vi "configuration UI.vi"() -> ()   [LabVIEW 2013, in "TEC editor node.lvclass"]
uses:
  TEC editor node.lvclass
  <vilib>/NI/Configuration Framework/Node/NodeRef.ctl
  <vilib>/NI/Configuration Framework/Node/NISE_CEF_Node.lvclass
  <vilib>/NI/AMC/Message Queue.ctl
  <vilib>/NI/AMC/Message.ctl
  <vilib>/NI/Tools/Keyed Array/KeyedArray.ctl
  <vilib>/NI/Configuration Framework/Node/UserEventRef.ctl
  <vilib>/NI/Configuration Framework/Controls/EventCluster.ctl
  <vilib>/NI/DCAF UI Toolkit/Controls/Move One Right.ctl
  <vilib>/NI/DCAF UI Toolkit/Controls/Move One Left.ctl
  configuration/TEC configuration.lvclass
  <vilib>/Utility/miscctls.llb/LVRowAndColumnTypeDef.ctl
  <vilib>/Utility/miscctls.llb/LVPositionTypeDef.ctl
  configuration/TEC configuration.lvclass/TEC configuration.ctl
  TEC editor node.lvclass/TEC editor node.ctl
  <vilib>/NI/Tag Bus/tag/Data Type.ctl
  <vilib>/NI/Tag Bus Module Framework/channel/channel classification.ctl
  <vilib>/NI/Tag Bus Module Framework/channel/TBM channel.lvclass/TBM channel.ctl
  <vilib>/NI/Configuration Framework/serializable configuration/NISE_CEF_serializable configuration.lvclass/NISE_CEF_serializable configuration.ctl
  <vilib>/NI/Tag Bus/tag/tag descriptor.lvclass/tag descriptor.ctl
  configuration/Write receive on port.vi
  configuration/Write send to port.vi
  configuration/Write send from port.vi
  configuration/Write send to address.vi
  configuration/Write estimated array size.vi
  configuration/Read receive on port.vi
  configuration/Read send from port.vi
  configuration/Read send to address.vi
  configuration/Read send to port.vi
  configuration/Read estimated array size.vi
  <vilib>/NI/DCAF/Tag Editor Core/Configuration Editor/Classes/Module editor node/Read display name.vi
  <vilib>/Utility/LVClass/Get LV Class Name.vi
  <vilib>/NI/Configuration Framework/error generator/NISE_error generator.vi
  <vilib>/NI/Configuration Framework/serializable configuration/NISE_CEF_serializable configuration.lvclass
  <vilib>/NI/DCAF/Tag Editor Core/Configuration Editor/Classes/Module editor node/module editor node.lvclass
  <vilib>/NI/Configuration Framework/NISE_CEF_TreeControl.lvlib
  <vilib>/NI/Tag Bus/tag/tag descriptor.lvclass
  <vilib>/NI/Module Execution Interface/Engine Configuration/engine configuration.lvclass
  <vilib>/NI/Tag Bus Module Framework/channel/TBM channel.lvclass
  <vilib>/NI/DCAF/Tag Editor Core/Configuration Editor/Classes/Engine Parent/Engine Parent Editor Node.lvclass
  <vilib>/NI/DCAF UI Toolkit/Controls/DCAF UI Elements.lvlib
  <vilib>/NI/Tools/Keyed Array/Tools_KeyedArray.lvlib
  <vilib>/NI/AMC/AMC.lvlib
panel:
  in  "Tab Control":T1(tab)
  out "Guid":string
  in  "unpair":bool
  out "Paired with":string
  in  "pair":bool
  in  "Pairing Options":i32(listbox)
  in  "Filtering":string
  in  "remove to":T2
  in  "add to":T3
  in  "toExtList":i32(listbox)
  in  "fromExternallist":i32(listbox)
  in  "avail tags":i32(listbox)=-1
  in  "Estimated Received Array Size (bytes)":u16
  in  "receive on port":u16
  in  "send from port":u16
  in  "send to address":string
  in  "send to port":u16
  in  "user event":T4
  in  "main queue":T5
  in  "node ref":T6
  # "UDP Port Settings"
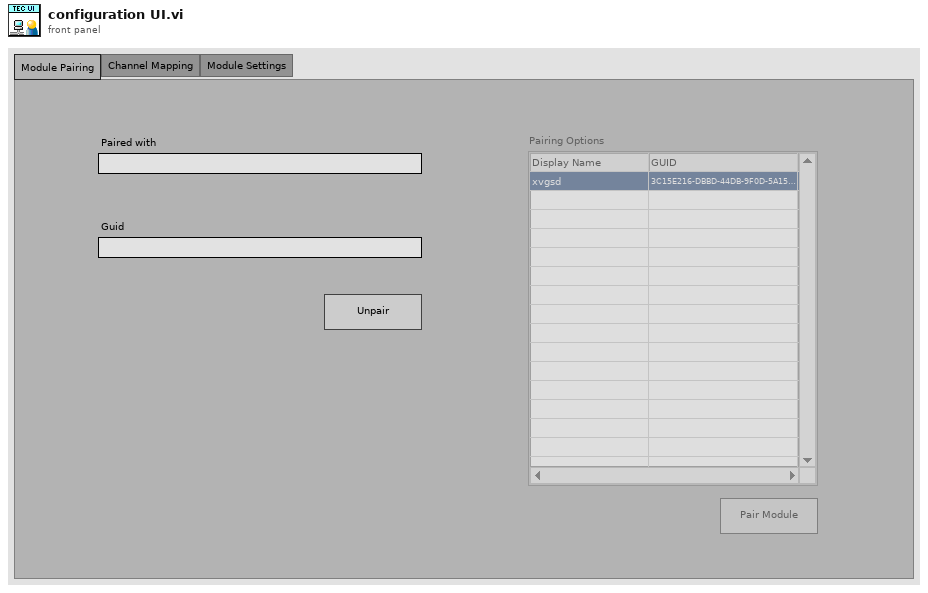
[diagram p1: front panel]
types:
  T1 = enum32{"Module Pairing", "Channel Mapping", "Module Settings"}
  T2 = typedef "DCAF UI Elements.lvlib/Move One Left.ctl" = bool
  T3 = typedef "DCAF UI Elements.lvlib/Move One Right.ctl" = bool
  T4 = typedef "NISE_CEF_Node.lvclass/UserEventRef.ctl" = refnum<user-event>
  T5 = typedef "AMC.lvlib/Message Queue.ctl" = refnum<queue>
  T6 = typedef "NISE_CEF_Node.lvclass/NodeRef.ctl" = refnum<data-value>
  T7 = typedef "LVPositionTypeDef.ctl" = cluster{"Left":i32, "Top":i32}
  T8 = typedef "LVRowAndColumnTypeDef.ctl" = cluster{"Row":i32, "Column":i32}
  T9 = typedef "NISE_CEF_TreeControl.lvlib/EventCluster.ctl" = cluster{"command":string, "data":string}
  T10 = typedef "TBM channel.lvclass/channel classification.ctl" = enum16{"input data", "output data", "processing parameter", "processing result"}
  T11 = typedef "tag bus.lvlib/tag descriptor.lvclass/Data Type.ctl" = enum16{"Double", "Single", "I64", "I32", "I16", "I8", "U64", "U32", "U16", "U8", "Boolean", "String", "Array of Double", "Array of Single", "Array of I64", "Array of I32", "Array of I16", "Array of I8", "Array of U64", "Array of U32", "Array of U16", "Array of U8", "Array of Boolean", "Array of String"}
  T12 = typedef "TEC editor node.lvclass/pair information.ctl" = cluster{"paired guid":string}
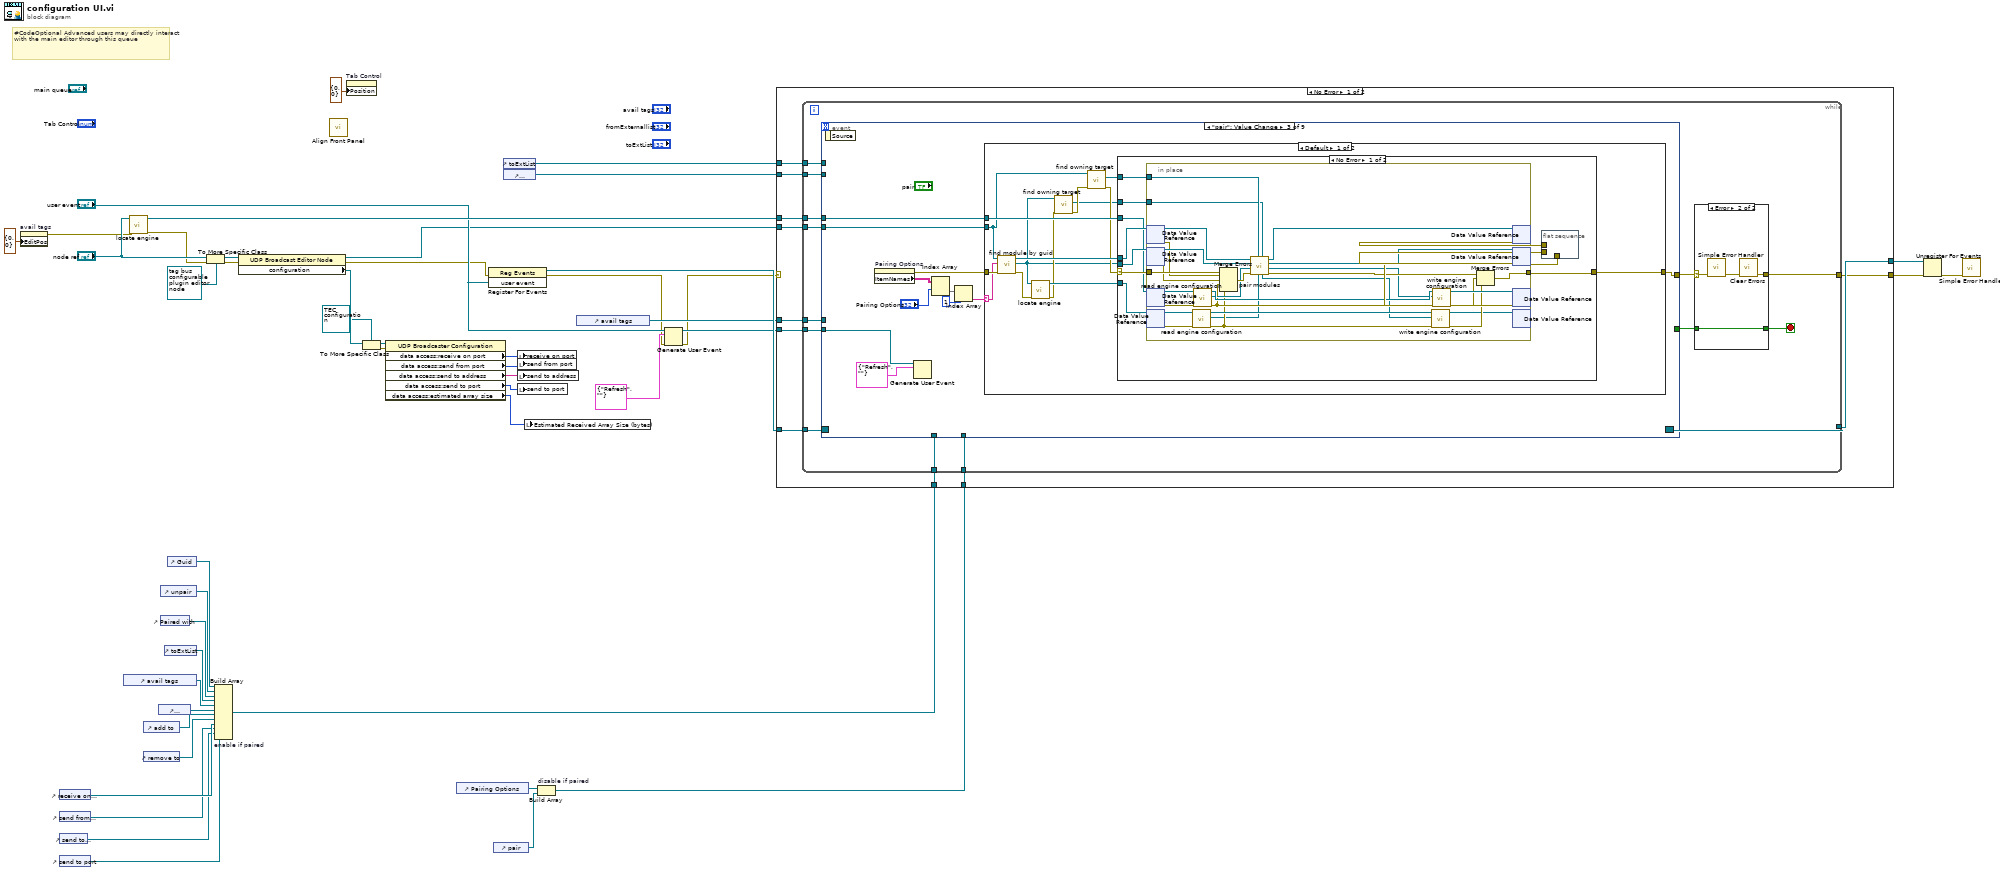
[diagram p0: block diagram]
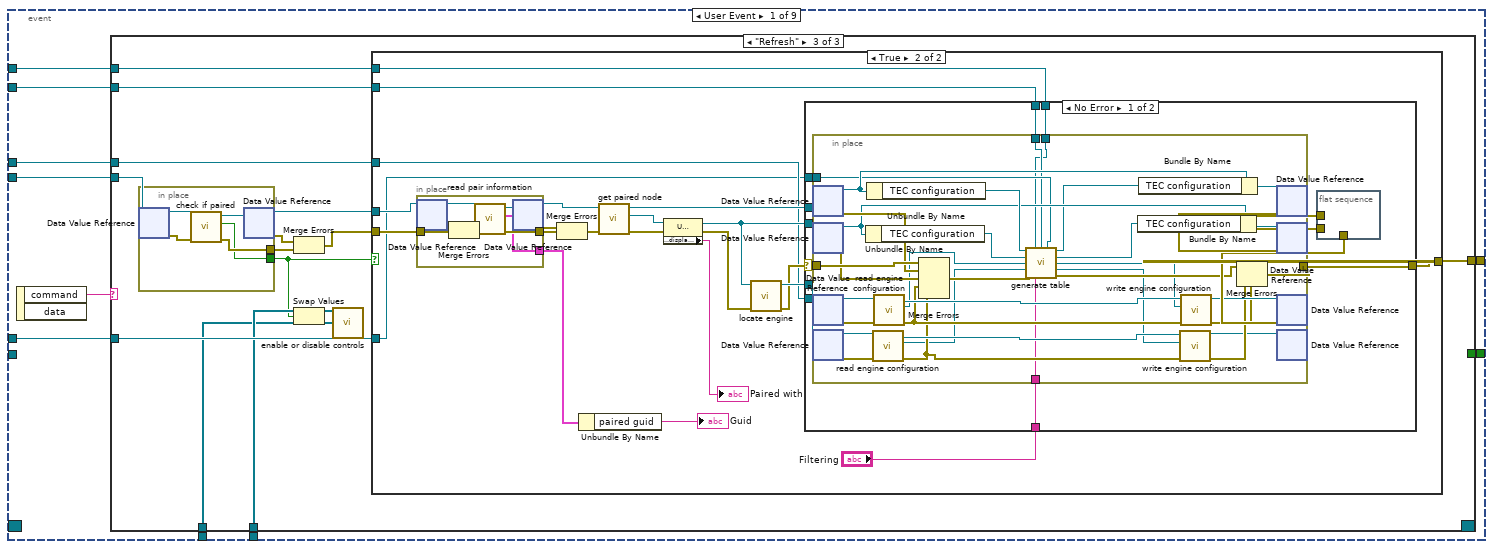
[diagram p3: hidden frame]
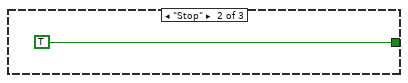
[diagram p5: hidden frame]
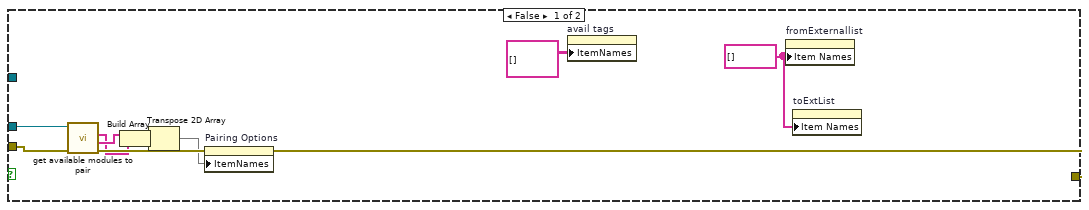
[diagram p6: hidden frame]
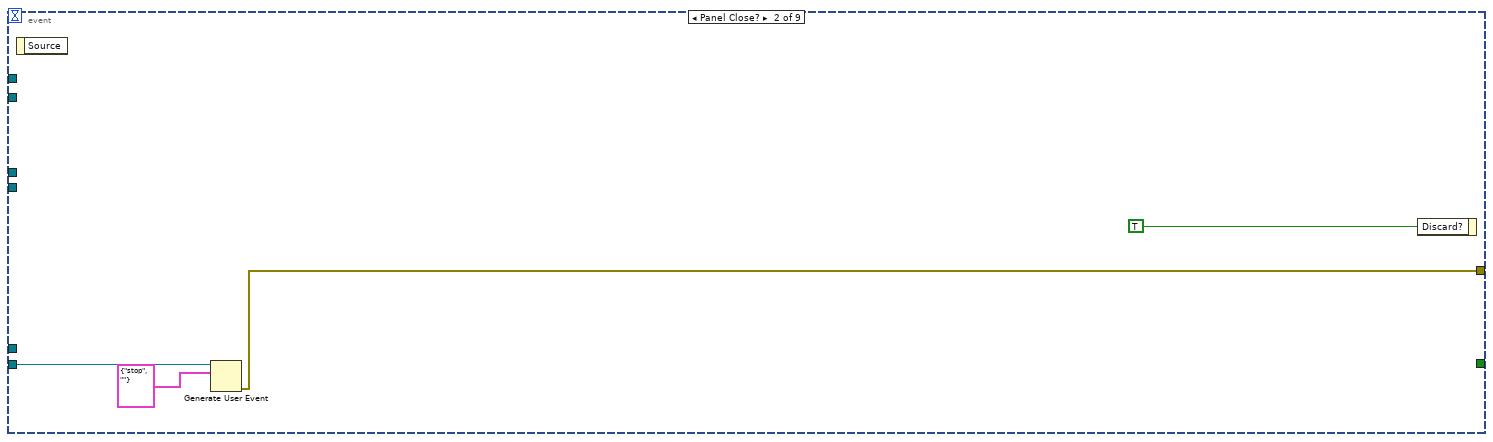
[diagram p8: hidden frame]
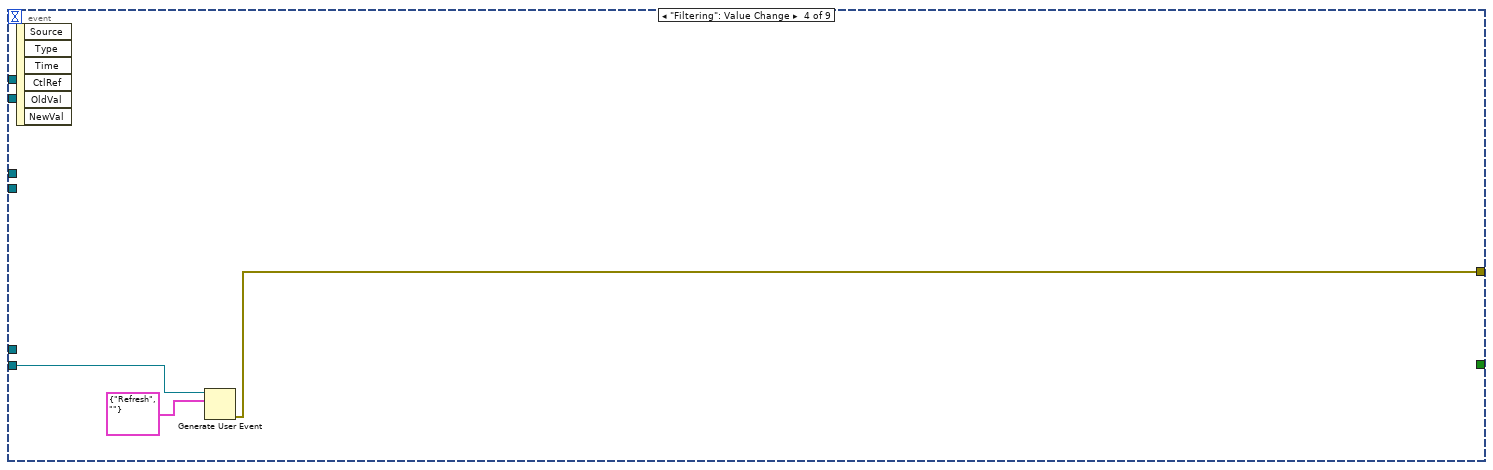
[diagram p11: hidden frame]
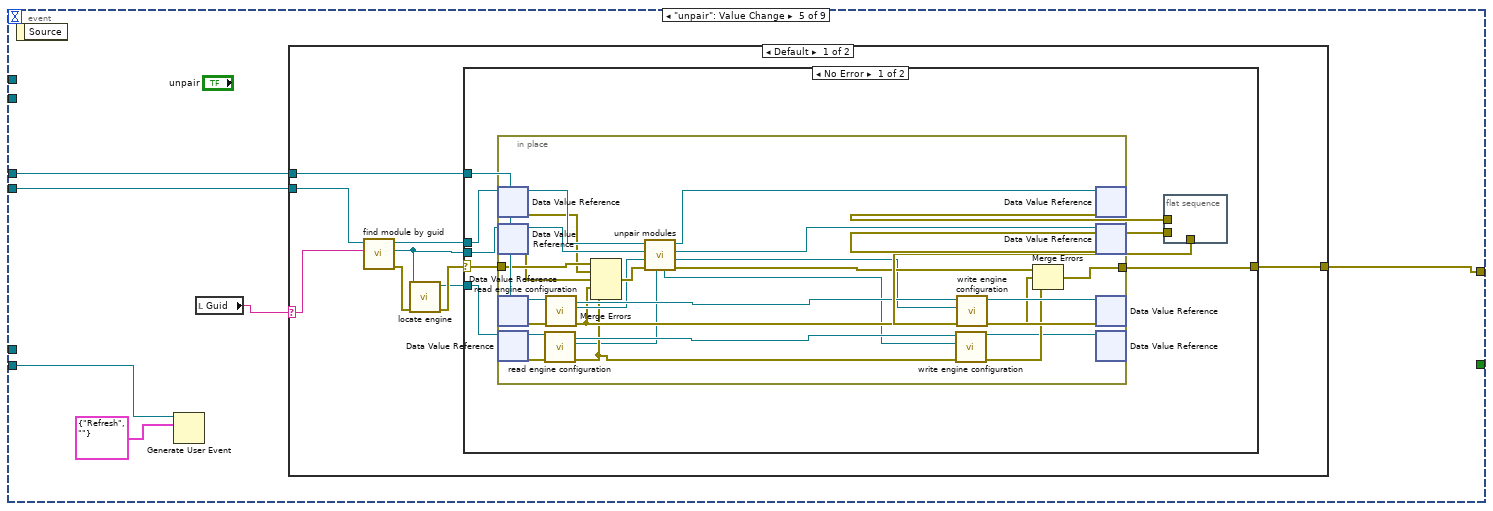
[diagram p12: hidden frame]
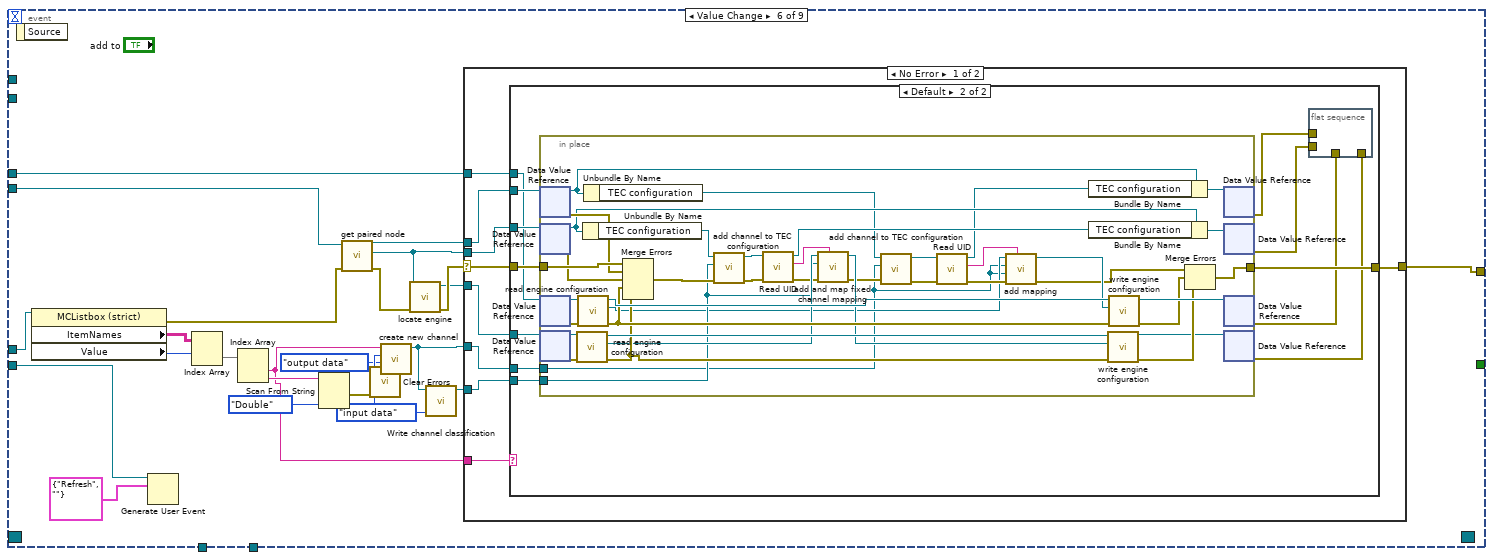
[diagram p15: hidden frame]
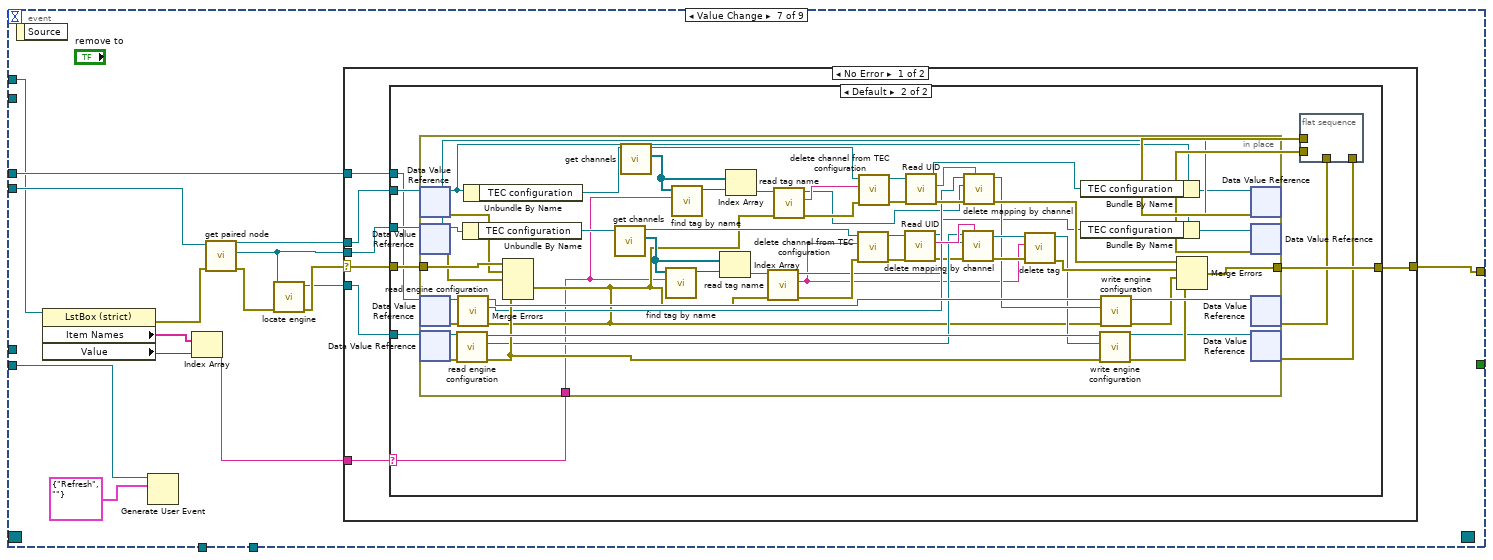
[diagram p18: hidden frame]
diagram:
  # "#CodeOptional Advanced users may directly interact with the main editor through this queue"
  n1 = property on="avail tags" class="MCListbox (strict)"("EditPos"=T8 {"Row"=0, "Column"=0} ("Edit Position")) -> (error out=w4:errorcluster)  [unwired: 2 in, 1 out]
  n2 = control-ref of="receive on port"() -> (w8:refnum<vi>)
  n3 = control-ref of="send from port"() -> (w7:refnum<vi>)
  n4 = control-ref of="send to address"() -> (w6:refnum<vi>)
  n5 = control-ref of="send to port"() -> (w5:refnum<vi>)
  n6 = control-ref of="avail tags"() -> (w29:refnum<vi>)
  n7 = call <vilib>:"locate engine.vi"("error in"=w4, "component"="node ref") -> ("error out"=w34:errorcluster, "engine"=w42:refnum<data-value>)  [unwired: 8 in]
  n8 = control-ref of="add to"() -> (w26:refnum<vi>)
  n9 = control-ref of="remove to"() -> (w27:refnum<vi>)
  n10 = control-ref of="fromExternallist"() -> (w28:refnum<vi>)
  n11 = control-ref of="unpair"() -> (w32:refnum<vi>)
  n12 = control-ref of="Paired with"() -> (w33:refnum<vi>)
  n13 = control-ref of="toExtList"() -> (w30:refnum<vi>)
  n14 = control-ref of="Guid"() -> (w31:refnum<vi>)
  n15 = To More Specific Class(target class=refnum<data-value> refnum ("data value reference"), reference="node ref", error in=w34) -> (specific class reference=w18:refnum<data-value>, error out=w44:errorcluster)
  n16 = Build Array "enable if paired"(w31, w32, w33, w30, w29, w28, w26, w27, w8, w7, w6, w5) -> (w24:refnum<vi>[])
  n17 = property class="UDP Broadcast Editor Node"(reference=w18, error in=w44) -> (reference out=w17:refnum<data-value>, error out=w19:errorcluster, "configuration"=w12:refnum<class "NISE_CEF_serializable configuration.lvclass">)
  n18 = call <vilib>:"Align Front Panel.vi"() -> ()  [unwired: 10 in, 2 out]
  n19 = property on="Tab Control" class="TabCtl (strict)"("Position"=T7 {"Left"=0, "Top"=0}) -> ()  [unwired: 2 in, 2 out]
  n20 = To More Specific Class(target class=refnum<class "TEC configuration.lvclass"> refnum ("UDP Broadcaster Configuration"), reference=w12) -> (specific class reference=w11:refnum<class "TEC configuration.lvclass">, error out=w10:errorcluster)  [unwired: 1 in]
  n21 = property class="UDP Broadcaster Configuration"(reference=w11, error in=w10) -> ("data access:receive on port"=w13:u16, "data access:send from port"=w14:u16, "data access:send to address"=w15:string, "data access:send to port"=w16:u16, "data access:estimated array size"=w2:u16)  [unwired: 2 out]
  n22 = control-ref of="Pairing Options"() -> (w25:refnum<vi>)
  n23 = register-events(error in=w19, "user event") -> (reference out=w48:refnum<event-registration>, error out=w21:errorcluster)  [unwired: 1 in]
  n24 = control-ref of="pair"() -> (w22:refnum<vi>)
  n25 = control-ref of="toExtList"() -> (w40:refnum<vi>)
  n26 = control-ref of="fromExternallist"() -> (w20:refnum<vi>)
  n27 = local write "receive on port"(w13) -> ()
  n28 = local write "send from port"(w14) -> ()
  n29 = local write "send to address"(w15) -> ()
  n30 = local write "send to port"(w16) -> ()
  n31 = local write "Estimated Received Array Size (bytes)"(w2) -> ()
  n32 = Build Array "disable if paired"(w25, w22) -> (w23:refnum<vi>[])
  n33 = control-ref of="avail tags"() -> (w41:refnum<vi>)
  n34 = Generate User Event(user event="user event", event data cluster=T9 {"command"="Refresh", "data"=""} ("event data"), error in=w21) -> (user event out=w38:T4, error out=w36:errorcluster)  [unwired: 1 in]
  n35 = case shown="No Error" w36 {
    selector: w36 -> [_ w540]
    tunnel: w48 -> [w59 w539]
    tunnel: [w58 w539] -> w47
    tunnel: [w57 w540] -> w46
    tunnel: w17 -> [w56 _]
    tunnel: w42 -> [w55 _]
    tunnel: w41 -> [w54 _]
    tunnel: w40 -> [w53 _]
    tunnel: w38 -> [w52 _]
    tunnel: w24 -> [w51 _]
    tunnel: w23 -> [w50 _]
    tunnel: w20 -> [w49 _]
    frame No Error {
      n36 = while {
        tunnel: w59 -> [w73]
        tunnel: [w72] -> w58
        tunnel: w56 -> [w67]
        tunnel: w55 -> [w66]
        tunnel: w52 -> [w65]
        tunnel: w54 -> [w64]
        tunnel: w53 -> [w63]
        tunnel: [w68] -> w57
        tunnel: w51 -> [w62]
        tunnel: w50 -> [w61]
        tunnel: w49 -> [w60]
        stop <- w70 stop-if-true
        n37 = event shown="[2] \"pair\": Value Change" {
          selector: w73 -> [_ _ _ _ _ _ _ _ _]
          dyn-events: [_ _ _ _ _ _ _ _ _] -> w72
          timeout: _ -> [_ _ _ _ _ _ _ _ _]
          tunnel: [w89 _ _ _ _ _ _ _ _] -> w69
          tunnel: [w87 w198 w205 w268 w275 w345 w424 w504 w531] -> w71
          tunnel: w67 -> [w86 _ w207 _ w276 w341 w420 w503 w530]
          tunnel: w66 -> [w85 _ w204 _ w274 w344 w423 _ _]
          tunnel: w65 -> [_ w199 w202 w269 w271 w336 w415 _ _]
          tunnel: w64 -> [w84 _ _ _ _ w330 _ _ _]
          tunnel: w63 -> [w83 _ _ _ _ _ w412 _ _]
          tunnel: w62 -> [w82 _ _ _ _ _ _ _ _]
          tunnel: w61 -> [w81 _ _ _ _ _ _ _ _]
          tunnel: w60 -> [w80 _ _ _ _ _ _ _ _]
          event User Event {
            n38 = event-data() -> ("command"=w88:string)  [unwired: 1 in, 1 out]
            n39 = case shown="\"Refresh\"" w88 {
              tunnel: [_ TRUE _] -> w89
              tunnel: [_ _ w102] -> w87
              tunnel: w86 -> [_ _ w101]
              tunnel: w85 -> [_ _ w103]
              tunnel: w84 -> [_ _ w105]
              tunnel: w83 -> [_ _ w104]
              tunnel: w82 -> [_ _ w95]
              tunnel: w81 -> [_ _ w96]
              tunnel: w80 -> [_ _ w91]
              frame Default {
              }
              frame "Stop" {
              }
              frame "Refresh" {
                n40 = in-place {
                  in-place-border: [w194] -> w98
                  in-place-border: [w193] -> w92
                  n41 = in-place-dvr #1(w101) -> (w197:refnum<class "TEC editor node.lvclass">, w195:errorcluster)
                  n42 = call "check if paired.vi"("error in"=w195, "UDP Broadcast Editor Node in"=w197) -> ("error out"=w194:errorcluster, "paired"=w193:bool, "UDP Broadcast Editor Node out"=w196:refnum<class "TEC editor node.lvclass">)  [unwired: 7 in]
                  n43 = in-place-dvr #1(w196) -> (w100:refnum<data-value>, w99:errorcluster)
                }
                n44 = Merge Errors(w99, w98) -> (w93:errorcluster)
                n45 = Swap Values(12:w96, 13:w92, 14:w95) -> (1:w97:refnum<vi>[], 3:w94:refnum<vi>[])
                n46 = call "enable or disable controls.vi"("disable set"=w94, "enable set"=w97) -> ()  [unwired: 10 in]
                n47 = case shown="True" w92 {
                  tunnel: w105 -> [_ w117]
                  tunnel: w104 -> [_ w118]
                  tunnel: w103 -> [_ w120]
                  tunnel: [w111 w124] -> w102
                  tunnel: w100 -> [w115 w127]
                  tunnel: w93 -> [w114 w128]
                  tunnel: w91 -> [_ w119]
                  frame False {
                    w106 = string[] [] ("Item Names")
                    n48 = call "get available modules to pair.vi"("error in"=w114, "editor in"=w115) -> ("error out"=w113:errorcluster, "Display Name"=w109:string[], "IDs"=w108:string[])  [unwired: 6 in, 1 out]
                    n49 = Build Array(w109, w108) -> (w112:string[][])
                    n50 = Transpose 2D Array(2D array=w112) -> (transposed array=w110:string[][])
                    n51 = property on="Pairing Options" class="MCListbox (strict)"(error in=w113, "ItemNames"=w110) -> (error out=w111:errorcluster)  [unwired: 1 in, 1 out]
                    n52 = property on="avail tags" class="MCListbox (strict)"("ItemNames"=string[][] [] ("Item Names")) -> ()  [unwired: 2 in, 2 out]
                    n53 = property on="fromExternallist" class="LstBox (strict)"("Item Names"=w106) -> ()  [unwired: 2 in, 2 out]
                    n54 = property on="toExtList" class="LstBox (strict)"("Item Names"=w106) -> ()  [unwired: 2 in, 2 out]
                  }
                  frame True {
                    n55 = in-place {
                      in-place-border: w128 -> [w188]
                      in-place-border: [w192] -> w135
                      in-place-border: [w186] -> w130
                      n56 = in-place-dvr #2(w127) -> (w191:refnum<class "TEC editor node.lvclass">, w187:errorcluster)
                      n57 = Merge Errors(w188, w187) -> (w189:errorcluster)
                      n58 = call "read pair information.vi"("error in"=w189, "UDP Broadcast Editor Node in"=w191) -> ("error out"=w192:errorcluster, "pair info"=w186:T12, "UDP Broadcast Editor Node out"=w190:refnum<class "TEC editor node.lvclass">)  [unwired: 7 in]
                      n59 = in-place-dvr #2(w190) -> (w137:refnum<data-value>, w134:errorcluster)
                    }
                    n60 = Merge Errors(w135, w134) -> (w136:errorcluster)
                    n61 = Unbundle By Name(w130) -> ("paired guid"=→"Guid":string)
                    n62 = call "get paired node.vi"("error in"=w136, "editor in"=w137) -> ("error out"=w132:errorcluster, "paired node"=w133:refnum<data-value>, "editor out"=w122:refnum<data-value>)  [unwired: 7 in]
                    n63 = property class="UDP Broadcast Editor Node"(reference=w133, error in=w132) -> (reference out=w121:refnum<data-value>, error out=w123:errorcluster, "Data Access:display name"=→"Paired with":string)
                    n64 = call <vilib>:"locate engine.vi"("error in"=w123, "component"=w121) -> ("error out"=w125:errorcluster, "engine"=w126:refnum<data-value>)  [unwired: 8 in]
                    n65 = case shown="No Error" w125 {
                      selector: w125 -> [w150 w185]
                      tunnel: [w149 w185] -> w124
                      tunnel: w126 -> [w145 _]
                      tunnel: w122 -> [w144 _]
                      tunnel: w121 -> [w143 _]
                      tunnel: w120 -> [w142 _]
                      tunnel: w119 -> [w141 _]
                      tunnel: w118 -> [w140 _]
                      tunnel: w117 -> [w139 _]
                      tunnel: "Filtering" -> [w138 _]
                      frame No Error {
                        n66 = in-place {
                          in-place-border: w150 -> [w184]
                          in-place-border: [w177] -> w149
                          in-place-border: w141 -> [w153]
                          in-place-border: w140 -> [w152]
                          in-place-border: w139 -> [w154]
                          in-place-border: w138 -> [w151]
                          n67 = in-place-dvr #3(w144) -> (w160:refnum<class "TEC editor node.lvclass">, w183:errorcluster)
                          n68 = in-place-dvr #4(w143) -> (w157:refnum<class "TEC editor node.lvclass">, w182:errorcluster)
                          n69 = in-place-dvr #5(w142) -> (w181:refnum<class "Engine Parent Editor Node.lvclass">, w180:errorcluster)
                          n70 = in-place-dvr #6(w145) -> (w173:refnum<class "Engine Parent Editor Node.lvclass">, w172:errorcluster)
                          n71 = Unbundle By Name(w157) -> ("TEC configuration"=w161:refnum<class "TEC configuration.lvclass">)
                          n72 = Unbundle By Name(w160) -> ("TEC configuration"=w162:refnum<class "TEC configuration.lvclass">)
                          n73 = call <vilib>:"read engine configuration.vi"("error in"=w172, "Engine Parent Editor Node in"=w173) -> ("error out"=w171:errorcluster, "engine configuration"=w164:refnum<class "engine configuration.lvclass">, "Engine Parent Editor Node out"=w174:refnum<class "Engine Parent Editor Node.lvclass">)  [unwired: 7 in]
                          n74 = call <vilib>:"read engine configuration.vi"("error in"=w180, "Engine Parent Editor Node in"=w181) -> ("error out"=w175:errorcluster, "engine configuration"=w163:refnum<class "engine configuration.lvclass">, "Engine Parent Editor Node out"=w179:refnum<class "Engine Parent Editor Node.lvclass">)  [unwired: 7 in]
                          n75 = Merge Errors(w184, w183, w182, w175, w171) -> (w168:errorcluster)
                          n76 = call "generate table.vi"("TEC in"=w162, "from TEC"=w152, "to TEC"=w153, "avail tags"=w154, "Pair in"=w161, "engine configuration in"=w163, "paired engine in"=w164, "error in"=w168, "Filtering"=w151) -> ("TEC out"=w155:refnum<class "TEC configuration.lvclass">, "pair out"=w156:refnum<class "TEC configuration.lvclass">, "engine configuration out"=w165:refnum<class "engine configuration.lvclass">, "paired engine out"=w166:refnum<class "engine configuration.lvclass">, "error out"=w167:errorcluster)  [unwired: 2 in]
                          n77 = Bundle By Name(cluster=w157, "TEC configuration"=w156) -> (w158:refnum<class "TEC editor node.lvclass">)
                          n78 = Bundle By Name(cluster=w160, "TEC configuration"=w155) -> (w159:refnum<class "TEC editor node.lvclass">)
                          n79 = call <vilib>:"write engine configuration.vi"("error in"=w171, "engine configuration"=w166, "Engine Parent Editor Node in"=w174) -> ("error out"=w170:errorcluster, "Engine Parent Editor Node out"=w169:refnum<class "Engine Parent Editor Node.lvclass">)  [unwired: 7 in]
                          n80 = call <vilib>:"write engine configuration.vi"("error in"=w175, "engine configuration"=w165, "Engine Parent Editor Node in"=w179) -> ("error out"=w176:errorcluster, "Engine Parent Editor Node out"=w178:refnum<class "Engine Parent Editor Node.lvclass">)  [unwired: 7 in]
                          n81 = Merge Errors(w167, w176, w170) -> (w177:errorcluster)
                          n82 = in-place-dvr #3(w159) -> (w148:errorcluster)  [unwired: 1 out]
                          n83 = in-place-dvr #4(w158) -> (w147:errorcluster)  [unwired: 1 out]
                          n84 = in-place-dvr #5(w178) -> (w146:errorcluster)  [unwired: 1 out]
                          n85 = in-place-dvr #6(w169) -> ()  [unwired: 2 out]
                        }
                        n86 = flat-sequence {
                          tunnel: w148 -> [_]
                          tunnel: w147 -> [_]
                          tunnel: w146 -> [_]
                          frame #0 {
                          }
                        }
                      }
                      frame Error {
                      }
                    }
                  }
                }
              }
            }
          }
          event Panel Close? {
            n87 = event-data() -> ()  [unwired: 1 in, 1 out]
            n88 = Generate User Event(user event=w199, event data cluster=T9 {"command"="stop", "data"=""} ("event data")) -> (error out=w198:errorcluster)  [unwired: 2 in, 1 out]
            n89 = event-data("Discard?"=TRUE) -> ()  [unwired: 1 in, 1 out]
          }
          event "pair": Value Change {
            n90 = event-data() -> ()  [unwired: 1 in, 1 out]
            n91 = property on="Pairing Options" class="MCListbox (strict)"() -> (error out=w206:errorcluster, "ItemNames"=w212:string[][])  [unwired: 2 in, 1 out]
            n92 = Generate User Event(user event=w202, event data cluster=T9 {"command"="Refresh", "data"=""} ("event data")) -> ()  [unwired: 2 in, 2 out]
            n93 = Index Array(array=w212, index (row)="Pairing Options") -> (element=w210:string[])  [unwired: 1 in]
            n94 = Index Array(array=w210, index=1) -> (element=w208:string)
            n95 = case shown="Default" w208 {
              selector: w208 -> [w225 _]
              tunnel: w207 -> [w216 _]
              tunnel: w206 -> [w226 w267]
              tunnel: [w224 w267] -> w205
              tunnel: w204 -> [w222 _]
              frame Default {
                n96 = call "find module by guid.vi"("error in (no error)"=w226, "GUID"=w225, "ME in"=w216) -> ("error out"=w221:errorcluster, "UDP refs"=w215:refnum<data-value>, "ME out"=w223:refnum<data-value>)  [unwired: 6 in]
                n97 = call <vilib>:"locate engine.vi"("error in"=w221, "component"=w215) -> ("error out"=w217:errorcluster, "engine"=w220:refnum<data-value>)  [unwired: 8 in]
                n98 = call "find owning target.vi"("error in"=w217, "node"=w215) -> ("error out"=w219:errorcluster, "target configuration"=w213:refnum<class "PL_Target Configuration.lvclass">)  [unwired: 7 in, 1 out]
                n99 = call "find owning target.vi"("error in"=w219, "node"=w216) -> ("error out"=w218:errorcluster, "target configuration"=w214:refnum<class "PL_Target Configuration.lvclass">)  [unwired: 7 in, 1 out]
                n100 = case shown="No Error" w218 {
                  selector: w218 -> [w237 w266]
                  tunnel: [w236 w266] -> w224
                  tunnel: w223 -> [w235 _]
                  tunnel: w215 -> [w234 _]
                  tunnel: w222 -> [w233 _]
                  tunnel: w220 -> [w229 _]
                  tunnel: w214 -> [w228 _]
                  tunnel: w213 -> [w227 _]
                  frame No Error {
                    n101 = in-place {
                      in-place-border: w237 -> [w265]
                      in-place-border: [w250] -> w236
                      in-place-border: w228 -> [w239]
                      in-place-border: w227 -> [w238]
                      n102 = in-place-dvr #7(w235) -> (w262:refnum<class "TEC editor node.lvclass">, w260:errorcluster)
                      n103 = in-place-dvr #8(w234) -> (w263:refnum<class "TEC editor node.lvclass">, w259:errorcluster)
                      n104 = in-place-dvr #9(w233) -> (w256:refnum<class "Engine Parent Editor Node.lvclass">, w255:errorcluster)
                      n105 = in-place-dvr #10(w229) -> (w246:refnum<class "Engine Parent Editor Node.lvclass">, w245:errorcluster)
                      n106 = call <vilib>:"read engine configuration.vi"("error in"=w245, "Engine Parent Editor Node in"=w246) -> ("error out"=w244:errorcluster, "engine configuration"=w240:refnum<class "engine configuration.lvclass">, "Engine Parent Editor Node out"=w247:refnum<class "Engine Parent Editor Node.lvclass">)  [unwired: 7 in]
                      n107 = call <vilib>:"read engine configuration.vi"("error in"=w255, "Engine Parent Editor Node in"=w256) -> ("error out"=w248:errorcluster, "engine configuration"=w252:refnum<class "engine configuration.lvclass">, "Engine Parent Editor Node out"=w254:refnum<class "Engine Parent Editor Node.lvclass">)  [unwired: 7 in]
                      n108 = Merge Errors(w265, w260, w259, w248, w244) -> (w261:errorcluster)
                      n109 = call "pair modules.vi"("Paired Target Configuration"=w238, "paired engine in"=w240, "Target Configuration"=w239, "error in"=w261, "engine configuration in"=w252, "module to pair with"=w263, "UDP Broadcast Editor Node in"=w262) -> ("error out"=w264:errorcluster, "engine configuration out"=w251:refnum<class "engine configuration.lvclass">, "module to pair with out"=w257:refnum<class "TEC editor node.lvclass">, "UDP Broadcast Editor Node out"=w258:refnum<class "TEC editor node.lvclass">, "paired engine out"=w241:refnum<class "engine configuration.lvclass">)
                      n110 = call <vilib>:"write engine configuration.vi"("error in"=w244, "engine configuration"=w241, "Engine Parent Editor Node in"=w247) -> ("error out"=w243:errorcluster, "Engine Parent Editor Node out"=w242:refnum<class "Engine Parent Editor Node.lvclass">)  [unwired: 7 in]
                      n111 = call <vilib>:"write engine configuration.vi"("error in"=w248, "engine configuration"=w251, "Engine Parent Editor Node in"=w254) -> ("error out"=w249:errorcluster, "Engine Parent Editor Node out"=w253:refnum<class "Engine Parent Editor Node.lvclass">)  [unwired: 7 in]
                      n112 = Merge Errors(w264, w249, w243) -> (w250:errorcluster)
                      n113 = in-place-dvr #7(w258) -> (w232:errorcluster)  [unwired: 1 out]
                      n114 = in-place-dvr #8(w257) -> (w231:errorcluster)  [unwired: 1 out]
                      n115 = in-place-dvr #9(w253) -> (w230:errorcluster)  [unwired: 1 out]
                      n116 = in-place-dvr #10(w242) -> ()  [unwired: 2 out]
                    }
                    n117 = flat-sequence {
                      tunnel: w232 -> [_]
                      tunnel: w231 -> [_]
                      tunnel: w230 -> [_]
                      frame #0 {
                      }
                    }
                  }
                  frame Error {
                  }
                }
              }
              frame "" {
                # "do nothing if nothing was selected"
              }
            }
          }
          event "Filtering": Value Change {
            n118 = event-data() -> ()  [unwired: 1 in, 6 out]
            n119 = Generate User Event(user event=w269, event data cluster=T9 {"command"="Refresh", "data"=""} ("event data")) -> (error out=w268:errorcluster)  [unwired: 2 in, 1 out]
          }
          event "unpair": Value Change {
            n120 = event-data() -> ()  [unwired: 1 in, 1 out]
            n121 = Generate User Event(user event=w271, event data cluster=T9 {"command"="Refresh", "data"=""} ("event data")) -> ()  [unwired: 2 in, 2 out]
            n122 = local read "Guid"() -> (w273:string)
            n123 = case shown="Default" w273 {
              selector: w273 -> [w284 _]
              tunnel: w276 -> [w285 _]
              tunnel: [w283 _] -> w275
              tunnel: w274 -> [w281 _]
              frame Default {
                n124 = call "find module by guid.vi"("GUID"=w284, "ME in"=w285) -> ("error out"=w280:errorcluster, "UDP refs"=w278:refnum<data-value>, "ME out"=w282:refnum<data-value>)  [unwired: 7 in]
                n125 = call <vilib>:"locate engine.vi"("error in"=w280, "component"=w278) -> ("error out"=w279:errorcluster, "engine"=w277:refnum<data-value>)  [unwired: 8 in]
                n126 = case shown="No Error" w279 {
                  selector: w279 -> [w294 w321]
                  tunnel: [w293 w321] -> w283
                  tunnel: w282 -> [w292 _]
                  tunnel: w278 -> [w291 _]
                  tunnel: w281 -> [w290 _]
                  tunnel: w277 -> [w286 _]
                  frame No Error {
                    n127 = in-place {
                      in-place-border: w294 -> [w320]
                      in-place-border: [w305] -> w293
                      n128 = in-place-dvr #11(w292) -> (w317:refnum<class "TEC editor node.lvclass">, w315:errorcluster)
                      n129 = in-place-dvr #12(w291) -> (w318:refnum<class "TEC editor node.lvclass">, w314:errorcluster)
                      n130 = in-place-dvr #13(w290) -> (w311:refnum<class "Engine Parent Editor Node.lvclass">, w310:errorcluster)
                      n131 = in-place-dvr #14(w286) -> (w301:refnum<class "Engine Parent Editor Node.lvclass">, w300:errorcluster)
                      n132 = call <vilib>:"read engine configuration.vi"("error in"=w300, "Engine Parent Editor Node in"=w301) -> ("error out"=w299:errorcluster, "engine configuration"=w295:refnum<class "engine configuration.lvclass">, "Engine Parent Editor Node out"=w302:refnum<class "Engine Parent Editor Node.lvclass">)  [unwired: 7 in]
                      n133 = call <vilib>:"read engine configuration.vi"("error in"=w310, "Engine Parent Editor Node in"=w311) -> ("error out"=w303:errorcluster, "engine configuration"=w307:refnum<class "engine configuration.lvclass">, "Engine Parent Editor Node out"=w309:refnum<class "Engine Parent Editor Node.lvclass">)  [unwired: 7 in]
                      n134 = Merge Errors(w320, w315, w314, w303, w299) -> (w316:errorcluster)
                      n135 = call "unpair modules.vi"("paired engine in"=w295, "error in"=w316, "engine configuration in"=w307, "module to unpair"=w318, "UDP Broadcast Editor Node in"=w317) -> ("error out"=w319:errorcluster, "engine configuration out"=w306:refnum<class "engine configuration.lvclass">, "unpaired module"=w312:refnum<class "TEC editor node.lvclass">, "UDP Broadcast Editor Node out"=w313:refnum<class "TEC editor node.lvclass">, "paired engine out"=w296:refnum<class "engine configuration.lvclass">)  [unwired: 2 in]
                      n136 = call <vilib>:"write engine configuration.vi"("error in"=w299, "engine configuration"=w296, "Engine Parent Editor Node in"=w302) -> ("error out"=w298:errorcluster, "Engine Parent Editor Node out"=w297:refnum<class "Engine Parent Editor Node.lvclass">)  [unwired: 7 in]
                      n137 = call <vilib>:"write engine configuration.vi"("error in"=w303, "engine configuration"=w306, "Engine Parent Editor Node in"=w309) -> ("error out"=w304:errorcluster, "Engine Parent Editor Node out"=w308:refnum<class "Engine Parent Editor Node.lvclass">)  [unwired: 7 in]
                      n138 = Merge Errors(w319, w304, w298) -> (w305:errorcluster)
                      n139 = in-place-dvr #11(w313) -> (w289:errorcluster)  [unwired: 1 out]
                      n140 = in-place-dvr #12(w312) -> (w288:errorcluster)  [unwired: 1 out]
                      n141 = in-place-dvr #13(w308) -> (w287:errorcluster)  [unwired: 1 out]
                      n142 = in-place-dvr #14(w297) -> ()  [unwired: 2 out]
                    }
                    n143 = flat-sequence {
                      tunnel: w289 -> [_]
                      tunnel: w288 -> [_]
                      tunnel: w287 -> [_]
                      frame #0 {
                      }
                    }
                  }
                  frame Error {
                  }
                }
              }
              frame "" {
                # "do nothing if nothing was selected"
              }
            }
          }
          event Value Change {
            n144 = event-data() -> ()  [unwired: 1 in, 1 out]
            n145 = property class="MCListbox (strict)"(reference=w330) -> (error out=w323:errorcluster, "ItemNames"=w335:string[][], "Value"=w334:i32)  [unwired: 1 in, 1 out]
            n146 = Generate User Event(user event=w336, event data cluster=T9 {"command"="Refresh", "data"=""} ("event data")) -> ()  [unwired: 2 in, 2 out]
            n147 = Index Array(array=w335, index (row)=w334) -> (element=w331:string[])  [unwired: 1 in]
            n148 = Index Array(array=w331) -> (element #1=w324:string, element #2=w333:string)  [unwired: 2 in]
            n149 = Scan From String(input string=w333, default 1=Data_Type."Double" ("data type")) -> (error out=w322:errorcluster, output 1=w329:T11)  [unwired: 3 in, 2 out]
            n150 = call "get paired node.vi"("error in"=w323, "editor in"=w341) -> ("error out"=w338:errorcluster, "paired node"=w339:refnum<data-value>, "editor out"=w340:refnum<data-value>)  [unwired: 7 in]
            n151 = call <vilib>:"Clear Errors.vi"("error in (no error)"=w322) -> ()  [unwired: 6 in, 1 out]
            n152 = call <vilib>:"create new channel.vi"("channel classification"=channel_classification."output data", "data type"=w329, "channel name"=w324) -> ("channel"=w327:refnum<class "TBM channel.lvclass">)  [unwired: 8 in]
            n153 = call <vilib>:"locate engine.vi"("error in"=w338, "component"=w339) -> ("error out"=w343:errorcluster, "engine"=w342:refnum<data-value>)  [unwired: 8 in]
            n154 = call <vilib>:"Write channel classification.vi"("channel classification"=channel_classification."input data", "channel in"=w327) -> ("channel out"=w326:refnum<class "TBM channel.lvclass">)  [unwired: 8 in, 1 out]
            n155 = case shown="No Error" w343 {
              selector: w343 -> [w354 w409]
              tunnel: [w353 w409] -> w345
              tunnel: w340 -> [w352 _]
              tunnel: w339 -> [w351 _]
              tunnel: w344 -> [w350 _]
              tunnel: w342 -> [w349 _]
              tunnel: w327 -> [w346 _]
              tunnel: w326 -> [w347 _]
              tunnel: w324 -> [w348 _]
              frame No Error {
                n156 = case shown="Default" w348 {
                  tunnel: w354 -> [w355 w367]
                  tunnel: [w355 w366] -> w353
                  tunnel: w352 -> [_ w365]
                  tunnel: w351 -> [_ w364]
                  tunnel: w350 -> [_ w363]
                  tunnel: w349 -> [_ w360]
                  tunnel: w347 -> [_ w357]
                  tunnel: w346 -> [_ w356]
                  frame "" {
                  }
                  frame Default {
                    n157 = in-place {
                      in-place-border: w367 -> [w408]
                      in-place-border: [w401] -> w366
                      in-place-border: w357 -> [w386]
                      in-place-border: w356 -> [w370]
                      n158 = in-place-dvr #15(w365) -> (w391:refnum<class "TEC editor node.lvclass">, w407:errorcluster)
                      n159 = in-place-dvr #16(w364) -> (w390:refnum<class "TEC editor node.lvclass">, w406:errorcluster)
                      n160 = in-place-dvr #17(w363) -> (w405:refnum<class "Engine Parent Editor Node.lvclass">, w404:errorcluster)
                      n161 = in-place-dvr #18(w360) -> (w397:refnum<class "Engine Parent Editor Node.lvclass">, w396:errorcluster)
                      n162 = call <vilib>:"read engine configuration.vi"("error in"=w396, "Engine Parent Editor Node in"=w397) -> ("error out"=w395:errorcluster, "engine configuration"=w387:refnum<class "engine configuration.lvclass">, "Engine Parent Editor Node out"=w398:refnum<class "Engine Parent Editor Node.lvclass">)  [unwired: 7 in]
                      n163 = call <vilib>:"read engine configuration.vi"("error in"=w404, "Engine Parent Editor Node in"=w405) -> ("error out"=w399:errorcluster, "engine configuration"=w372:refnum<class "engine configuration.lvclass">, "Engine Parent Editor Node out"=w403:refnum<class "Engine Parent Editor Node.lvclass">)  [unwired: 7 in]
                      n164 = Unbundle By Name(w390) -> ("TEC configuration"=w388:refnum<class "TEC configuration.lvclass">)
                      n165 = Unbundle By Name(w391) -> ("TEC configuration"=w378:refnum<class "TEC configuration.lvclass">)
                      n166 = Merge Errors(w408, w407, w406, w399, w395) -> (w392:errorcluster)
                      n167 = call "add channel to TEC configuration.vi"("error in"=w392, "channel"=w386, "TEC configuration in"=w388) -> ("error out"=w385:errorcluster, "TEC configuration out"=w384:refnum<class "TEC configuration.lvclass">)  [unwired: 7 in]
                      n168 = call <vilib>:"Read UID.vi"("error in"=w385, "configuration in"=w384) -> ("error out"=w383:errorcluster, "instance id"=w382:string, "configuration out"=w381:refnum<class "TEC configuration.lvclass">)  [unwired: 7 in]
                      n169 = call <vilib>:"add and map fixed channel mapping.vi"("module instance"=w382, "error in"=w383, "fixed channel"=w386, "engine configuration in"=w387) -> ("error out"=w379:errorcluster, "engine configuration out"=w380:refnum<class "engine configuration.lvclass">)  [unwired: 6 in]
                      n170 = call "add channel to TEC configuration.vi"("error in"=w379, "channel"=w370, "TEC configuration in"=w378) -> ("error out"=w376:errorcluster, "TEC configuration out"=w377:refnum<class "TEC configuration.lvclass">)  [unwired: 7 in]
                      n171 = call <vilib>:"Read UID.vi"("error in"=w376, "configuration in"=w377) -> ("error out"=w375:errorcluster, "instance id"=w371:string, "configuration out"=w374:refnum<class "TEC configuration.lvclass">)  [unwired: 7 in]
                      n172 = call <vilib>:"add mapping.vi"("owner ID"=w371, "error in"=w375, "channel"=w370, "tag descriptor"=w370, "engine configuration"=w372) -> ("error out"=w369:errorcluster, "engine configuration out"=w373:refnum<class "engine configuration.lvclass">)  [unwired: 5 in]
                      n173 = Bundle By Name(cluster=w391, "TEC configuration"=w374) -> (w368:refnum<class "TEC editor node.lvclass">)
                      n174 = Bundle By Name(cluster=w390, "TEC configuration"=w381) -> (w389:refnum<class "TEC editor node.lvclass">)
                      n175 = call <vilib>:"write engine configuration.vi"("error in"=w395, "engine configuration"=w380, "Engine Parent Editor Node in"=w398) -> ("error out"=w394:errorcluster, "Engine Parent Editor Node out"=w393:refnum<class "Engine Parent Editor Node.lvclass">)  [unwired: 7 in]
                      n176 = call <vilib>:"write engine configuration.vi"("error in"=w399, "engine configuration"=w373, "Engine Parent Editor Node in"=w403) -> ("error out"=w400:errorcluster, "Engine Parent Editor Node out"=w402:refnum<class "Engine Parent Editor Node.lvclass">)  [unwired: 7 in]
                      n177 = Merge Errors(w369, w400, w394) -> (w401:errorcluster)
                      n178 = in-place-dvr #15(w368) -> (w362:errorcluster)  [unwired: 1 out]
                      n179 = in-place-dvr #16(w389) -> (w361:errorcluster)  [unwired: 1 out]
                      n180 = in-place-dvr #17(w402) -> (w359:errorcluster)  [unwired: 1 out]
                      n181 = in-place-dvr #18(w393) -> (w358:errorcluster)  [unwired: 1 out]
                    }
                    n182 = flat-sequence {
                      tunnel: w362 -> [_]
                      tunnel: w361 -> [_]
                      tunnel: w359 -> [_]
                      tunnel: w358 -> [_]
                      frame #0 {
                      }
                    }
                  }
                }
              }
              frame Error {
              }
            }
          }
          event Value Change {
            n183 = event-data() -> ()  [unwired: 1 in, 1 out]
            n184 = property class="LstBox (strict)"(reference=w412) -> (error out=w411:errorcluster, "Item Names"=w414:string[], "Value"=w413:i32)  [unwired: 1 in, 1 out]
            n185 = Generate User Event(user event=w415, event data cluster=T9 {"command"="Refresh", "data"=""} ("event data")) -> ()  [unwired: 2 in, 2 out]
            n186 = Index Array(array=w414, index=w413) -> (element=w410:string)
            n187 = call "get paired node.vi"("error in"=w411, "editor in"=w420) -> ("error out"=w417:errorcluster, "paired node"=w418:refnum<data-value>, "editor out"=w419:refnum<data-value>)  [unwired: 7 in]
            n188 = call <vilib>:"locate engine.vi"("error in"=w417, "component"=w418) -> ("error out"=w422:errorcluster, "engine"=w421:refnum<data-value>)  [unwired: 8 in]
            n189 = case shown="No Error" w422 {
              selector: w422 -> [w431 w499]
              tunnel: [w430 w499] -> w424
              tunnel: w419 -> [w429 _]
              tunnel: w418 -> [w428 _]
              tunnel: w423 -> [w427 _]
              tunnel: w421 -> [w426 _]
              tunnel: w410 -> [w425 _]
              frame No Error {
                n190 = case shown="Default" w425 {
                  selector: w425 -> [_ w433]
                  tunnel: w431 -> [w432 w443]
                  tunnel: [w432 w442] -> w430
                  tunnel: w429 -> [_ w441]
                  tunnel: w428 -> [_ w440]
                  tunnel: w427 -> [_ w439]
                  tunnel: w426 -> [_ w436]
                  frame "" {
                  }
                  frame Default {
                    n191 = in-place {
                      in-place-border: w443 -> [w498]
                      in-place-border: [w491] -> w442
                      in-place-border: w433 -> [w445]
                      n192 = in-place-dvr #19(w441) -> (w483:refnum<class "TEC editor node.lvclass">, w497:errorcluster)
                      n193 = in-place-dvr #20(w440) -> (w482:refnum<class "TEC editor node.lvclass">, w496:errorcluster)
                      n194 = in-place-dvr #21(w439) -> (w495:refnum<class "Engine Parent Editor Node.lvclass">, w494:errorcluster)
                      n195 = in-place-dvr #22(w436) -> (w488:refnum<class "Engine Parent Editor Node.lvclass">, w487:errorcluster)
                      n196 = call <vilib>:"read engine configuration.vi"("error in"=w487, "Engine Parent Editor Node in"=w488) -> ("error out"=w486:errorcluster, "engine configuration"=w468:refnum<class "engine configuration.lvclass">, "Engine Parent Editor Node out"=w489:refnum<class "Engine Parent Editor Node.lvclass">)  [unwired: 7 in]
                      n197 = call <vilib>:"read engine configuration.vi"("error in"=w494, "Engine Parent Editor Node in"=w495) -> ("error out"=w451:errorcluster, "engine configuration"=w467:refnum<class "engine configuration.lvclass">, "Engine Parent Editor Node out"=w493:refnum<class "Engine Parent Editor Node.lvclass">)  [unwired: 7 in]
                      n198 = Unbundle By Name(w482) -> ("TEC configuration"=w458:refnum<class "TEC configuration.lvclass">)
                      n199 = Unbundle By Name(w483) -> ("TEC configuration"=w456:refnum<class "TEC configuration.lvclass">)
                      n200 = Merge Errors(w498, w497, w496, w451, w486) -> ()  [unwired: 1 out]
                      n201 = call-dynamic "get channels.vi"("TEC configuration in"=w458) -> ("channels"=w460:refnum<class "TBM channel.lvclass">[], "TEC configuration out"=w457:refnum<class "TEC configuration.lvclass">)  [unwired: 9 in]
                      n202 = call-dynamic "get channels.vi"("TEC configuration in"=w456) -> ("channels"=w463:refnum<class "TBM channel.lvclass">[], "TEC configuration out"=w455:refnum<class "TEC configuration.lvclass">)  [unwired: 9 in]
                      n203 = call <vilib>:"find tag by name.vi"("name"=w445, "tags in"=w460) -> ("index"=w459:i32)  [unwired: 9 in]
                      n204 = call <vilib>:"find tag by name.vi"("name"=w445, "tags in"=w463) -> ("index"=w462:i32)  [unwired: 9 in]
                      n205 = Index Array(array=w460, index=w459) -> (element=w461:refnum<class "TBM channel.lvclass">)
                      n206 = Index Array(array=w463, index=w462) -> (element=w464:refnum<class "TBM channel.lvclass">)
                      n207 = call <vilib>:"read tag name.vi"("error in"=w451, "system tag in"=w461) -> ("error out"=w452:errorcluster, "name"=w446:string, "system tag out"=w448:refnum<class "TBM channel.lvclass">)  [unwired: 7 in]
                      n208 = call <vilib>:"read tag name.vi"("error in"=w451, "system tag in"=w464) -> ("error out"=w453:errorcluster, "name"=w454:string, "system tag out"=w449:refnum<class "TBM channel.lvclass">)  [unwired: 7 in]
                      n209 = call "delete channel from TEC configuration.vi"("error in"=w452, "channel to delete"=w446, "TEC configuration in"=w457) -> ("error out"=w450:errorcluster, "TEC configuration out"=w477:refnum<class "TEC configuration.lvclass">)  [unwired: 7 in]
                      n210 = call "delete channel from TEC configuration.vi"("error in"=w453, "channel to delete"=w454, "TEC configuration in"=w455) -> ("error out"=w479:errorcluster, "TEC configuration out"=w480:refnum<class "TEC configuration.lvclass">)  [unwired: 7 in]
                      n211 = call <vilib>:"Read UID.vi"("error in"=w450, "configuration in"=w477) -> ("error out"=w447:errorcluster, "instance id"=w474:string, "configuration out"=w465:refnum<class "TEC configuration.lvclass">)  [unwired: 7 in]
                      n212 = call <vilib>:"Read UID.vi"("error in"=w479, "configuration in"=w480) -> ("error out"=w478:errorcluster, "instance id"=w473:string, "configuration out"=w466:refnum<class "TEC configuration.lvclass">)  [unwired: 7 in]
                      n213 = call <vilib>:"delete mapping by channel.vi"("owner ID"=w474, "error in"=w447, "channel"=w448, "engine configuration in"=w468) -> ("error out"=w475:errorcluster, "engine configuration out"=w476:refnum<class "engine configuration.lvclass">)  [unwired: 6 in]
                      n214 = call <vilib>:"delete mapping by channel.vi"("owner ID"=w473, "error in"=w478, "channel"=w449, "engine configuration in"=w467) -> ("error out"=w471:errorcluster, "engine configuration out"=w470:refnum<class "engine configuration.lvclass">)  [unwired: 6 in]
                      n215 = call <vilib>:"delete tag.vi"("error in"=w475, "tag name"=w446, "engine configuration in"=w476) -> ("error out"=w472:errorcluster, "engine configuration out"=w469:refnum<class "engine configuration.lvclass">)  [unwired: 7 in]
                      n216 = Bundle By Name(cluster=w483, "TEC configuration"=w466) -> (w444:refnum<class "TEC editor node.lvclass">)
                      n217 = Bundle By Name(cluster=w482, "TEC configuration"=w465) -> (w481:refnum<class "TEC editor node.lvclass">)
                      n218 = call <vilib>:"write engine configuration.vi"("error in"=w486, "engine configuration"=w469, "Engine Parent Editor Node in"=w489) -> ("error out"=w485:errorcluster, "Engine Parent Editor Node out"=w484:refnum<class "Engine Parent Editor Node.lvclass">)  [unwired: 7 in]
                      n219 = call <vilib>:"write engine configuration.vi"("error in"=w451, "engine configuration"=w470, "Engine Parent Editor Node in"=w493) -> ("error out"=w490:errorcluster, "Engine Parent Editor Node out"=w492:refnum<class "Engine Parent Editor Node.lvclass">)  [unwired: 7 in]
                      n220 = Merge Errors(w471, w472, w490, w485) -> (w491:errorcluster)
                      n221 = in-place-dvr #19(w444) -> (w438:errorcluster)  [unwired: 1 out]
                      n222 = in-place-dvr #20(w481) -> (w437:errorcluster)  [unwired: 1 out]
                      n223 = in-place-dvr #21(w492) -> (w435:errorcluster)  [unwired: 1 out]
                      n224 = in-place-dvr #22(w484) -> (w434:errorcluster)  [unwired: 1 out]
                    }
                    n225 = flat-sequence {
                      tunnel: w438 -> [_]
                      tunnel: w437 -> [_]
                      tunnel: w435 -> [_]
                      tunnel: w434 -> [_]
                      frame #0 {
                      }
                    }
                  }
                }
              }
              frame Error {
              }
            }
          }
          event "receive on port", "send from port", "send to address", "send to port": Value Change {
            n226 = event-data() -> ()  [unwired: 1 in, 6 out]
            n227 = call "get paired node.vi"("editor in"=w503) -> ("error out"=w500:errorcluster, "paired node"=w501:refnum<data-value>, "editor out"=w502:refnum<data-value>)  [unwired: 8 in]
            n228 = case shown="No Error" w500 {
              selector: w500 -> [_ w527]
              tunnel: [w509 w527] -> w504
              tunnel: w502 -> [w508 _]
              tunnel: w501 -> [w507 _]
              frame No Error {
                n229 = in-place {
                  in-place-border: [w518] -> w509
                  n230 = in-place-dvr #23(w508) -> (w526:refnum<class "TEC editor node.lvclass">, w521:errorcluster)
                  n231 = in-place-dvr #24(w507) -> (w514:refnum<class "TEC editor node.lvclass">, w512:errorcluster)
                  n232 = Unbundle By Name(w526) -> ("TEC configuration"=w525:refnum<class "TEC configuration.lvclass">)
                  n233 = Unbundle By Name(w514) -> ("TEC configuration"=w516:refnum<class "TEC configuration.lvclass">)
                  n234 = property class="UDP Broadcaster Configuration"(reference=w525, error in=w521, "data access:receive on port"="receive on port", "data access:send from port"="send from port", "data access:send to address"="send to address", "data access:send to port"="send to port") -> (reference out=w524:refnum<class "TEC configuration.lvclass">, error out=w522:errorcluster)
                  n235 = property class="UDP Broadcaster Configuration"(reference=w516, error in=w512, "data access:receive on port"="send to port", "data access:send to port"="receive on port") -> (reference out=w517:refnum<class "TEC configuration.lvclass">, error out=w513:errorcluster)
                  n236 = Bundle By Name(cluster=w526, "TEC configuration"=w524) -> (w523:refnum<class "TEC editor node.lvclass">)
                  n237 = Bundle By Name(cluster=w514, "TEC configuration"=w517) -> (w515:refnum<class "TEC editor node.lvclass">)
                  n238 = Merge Errors(w522, w513) -> (w518:errorcluster)
                  n239 = in-place-dvr #23(w523) -> (w505:errorcluster)  [unwired: 1 out]
                  n240 = in-place-dvr #24(w515) -> (w506:errorcluster)  [unwired: 1 out]
                }
                n241 = flat-sequence {
                  tunnel: w506 -> [_]
                  tunnel: w505 -> [_]
                  frame #0 {
                  }
                }
              }
              frame Error {
              }
            }
          }
          event "Estimated Received Array Size (bytes)": Value Change {
            n242 = event-data() -> ()  [unwired: 1 in, 6 out]
            n243 = in-place {
              in-place-border: [w533] -> w531
              in-place-border: "Estimated Received Array Size (bytes)" -> [w532]
              n244 = in-place-dvr #25(w530) -> (w535:refnum<class "TEC editor node.lvclass">, w534:errorcluster)
              n245 = Unbundle By Name(w535) -> ("TEC configuration"=w537:refnum<class "TEC configuration.lvclass">)
              n246 = property class="UDP Broadcaster Configuration"(reference=w537, error in=w534, "data access:estimated array size"=w532) -> (reference out=w538:refnum<class "TEC configuration.lvclass">, error out=w533:errorcluster)
              n247 = Bundle By Name(cluster=w535, "TEC configuration"=w538) -> (w536:refnum<class "TEC editor node.lvclass">)
              n248 = in-place-dvr #25(w536) -> (w529:errorcluster)  [unwired: 1 out]
            }
            n249 = flat-sequence {
              tunnel: w529 -> [_]
              frame #0 {
              }
            }
          }
        }
        n250 = case shown="Error" w71 {
          selector: w71 -> [w74 w78]
          tunnel: [w75 w79] -> w70
          tunnel: w69 -> [w75 w79]
          tunnel: [w74 w76] -> w68
          frame No Error {
          }
          frame Error {
            n251 = call <vilib>:"Simple Error Handler.vi"("error in (no error)"=w78) -> ("error out"=w77:errorcluster)  [unwired: 4 in, 4 out]
            n252 = call <vilib>:"Clear Errors.vi"("error in (no error)"=w77) -> ("error out"=w76:errorcluster)  [unwired: 6 in]
          }
        }
      }
    }
    frame Error {
    }
  }
  n253 = Unregister For Events(event registration refnum=w47, error in=w46) -> (error out=w43:errorcluster)
  n254 = call <vilib>:"Simple Error Handler.vi"("error in (no error)"=w43) -> ()  [unwired: 4 in, 5 out]
